vi "ERW-IoT Host Draft.vi"() -> ()   [LabVIEW 2026]
panel:
  out "data out 2":string
  out "data out":string
  out "connection ID":refnum<k5>
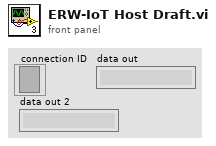
[diagram p1: front panel]
types:
  T1 = enum16{"Standard", "Buffered", "CRLF", "Immediate"}
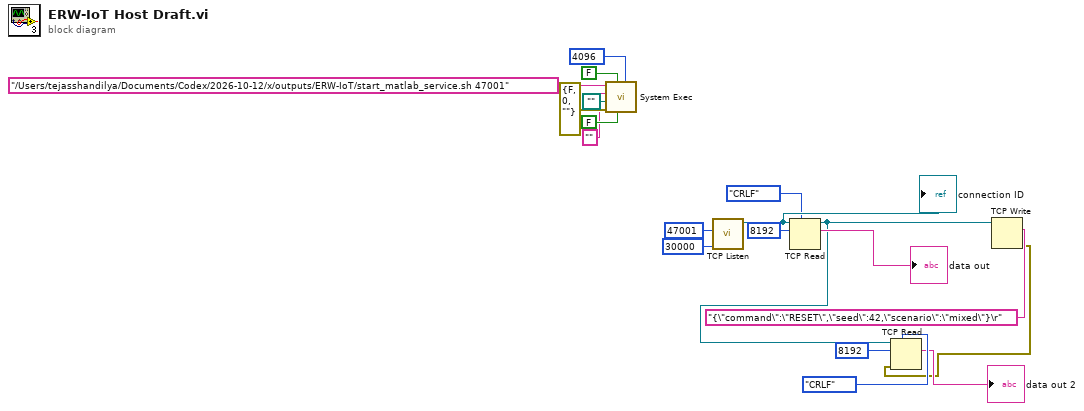
[diagram p0: block diagram]
diagram:
  n1 = call <vilib>:"System Exec.vi"("expected output size  (4096)"=u32 4096, "run minimized? (F)"=FALSE, "wait until completion? (T)"=FALSE, "error in (no error)"=errorcluster {"status"=FALSE, "code"=0, "source"=""}, "working directory"=path "", "standard input"="", "command line"="/Users/tejasshandilya/Documents/Codex/2026-10-12/x/outputs/ERW-IoT/start_matlab_service.sh 47001") -> ()  [unwired: 1 in, 4 out]
  n2 = call <vilib>:"TCP Listen.vi"("timeout ms (wait forever: -1)"=30000, "port"=u16 47001) -> ("connection ID"=w10:refnum<k5>)  [unwired: 5 in, 4 out]
  "connection ID" <- w10
  n3 = TCP Read(connection ID=w10, bytes to read=8192, 7:T1."CRLF" ("mode (standard)")) -> (connection ID out=w7:refnum<k5>, data out=→"data out":string)  [unwired: 2 in, 1 out]
  n4 = TCP Write(connection ID=w7, data in="{\"command\":\"RESET\",\"seed\":42,\"scenario\":\"mixed\"}\r") -> (error out=w2:errorcluster)  [unwired: 2 in, 2 out]
  n5 = TCP Read(connection ID=w7, bytes to read=8192, error in (no error)=w2, 7:T1."CRLF" ("mode (standard)")) -> (data out=→"data out 2":string)  [unwired: 1 in, 2 out]
